vi "MW_resource_name.vi"() -> ()   [LabVIEW 2025]
panel:
  in  "resource name":refnum<k15>="PXI1Slot2"
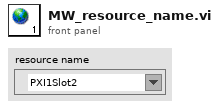
[diagram p1: front panel]
diagram:
